vi "FuncVI-probe.vi"(5 "InstanceRef":T2, 9 "arg list":T1[](array[typedef])) -> (0 "error out":bool, 3 "result":T1)   [LabVIEW 2021]
doc: "::: CalcExpress Toolkit :::\nCopyright (c) 2000-2026 Konstantin Shifershteyn. All rights reserved."
uses:
  cetypes.llb/CalcExpress Function Argument Info.ctl
  cetypes.llb/CalcExpress Instance RefNum.ctl
panel:
  in  "max arg num":i32=4
  in  "min arg num":i32=1
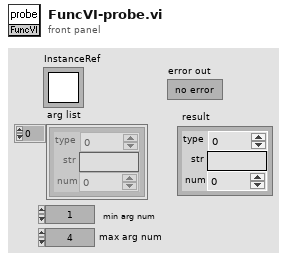
[diagram p1: front panel]
types:
  T1 = typedef "CalcExpress Function Argument Info.ctl" = cluster{"type":u32, "str":string, "num":dbl}
  T2 = typedef "CalcExpress Instance RefNum.ctl" = refnum<k1>
  T3 = cluster{"index":i32, "data type":enum32{"String", "DBL Number", "identifier", "1D Array of DBL", "2D Array of DBL", "CDB Number", "1D Array of CDB", "2D Array of CDB", "1D Array of String", "2D Array of String", "Unknown data type"}, "default num":dbl, "default str":string}[]
  T4 = cluster{"index":i32, "data type":enum32{"String", "DBL Number", "identifier", "1D Array of DBL", "2D Array of DBL", "CDB Number", "1D Array of CDB", "2D Array of CDB", "1D Array of String", "2D Array of String", "Unknown data type"}, "default num":dbl, "default str":string}
  T5 = cluster{"index":i32, "any type":i32, "default num":dbl, "default str":string}
  T6 = cluster{"data type":enum32{"String", "DBL Number", "identifier", "1D Array of DBL", "2D Array of DBL", "CDB Number", "1D Array of CDB", "2D Array of CDB", "1D Array of String", "2D Array of String", "Unknown data type"}, "str":string, "num":dbl}
  T7 = cluster{"index":i32, "data type":u32, "default num":dbl, "default str":string}[]
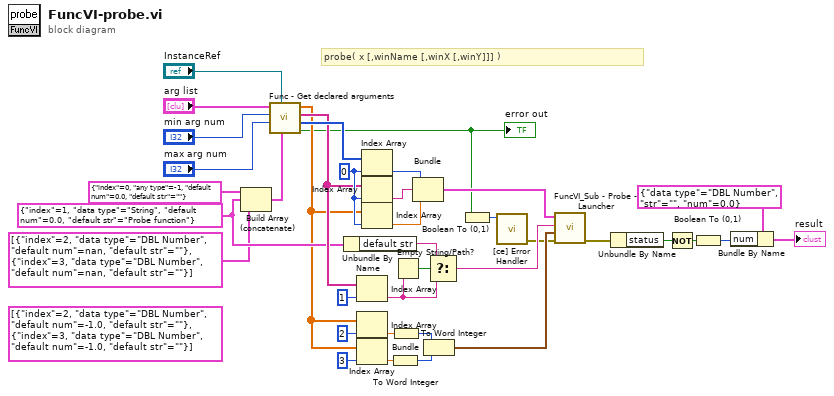
[diagram p0: block diagram]
diagram:
  (unwired) T3 [{"index"=2, "data type"=enum."DBL Number", "default num"=-1.0, "default str"=""}, {"index"=3, "data type"=enum."DBL Number", "default num"=-1.0, "default str"=""}]
  w29 = 0
  w23 = T4 {"index"=1, "data type"=enum."String", "default num"=0.0, "default str"="Probe function"} ("arg descriptor")
  # "probe( x [,winName [,winX [,winY]]] )"
  n1 = Build Array (concatenate)(T5 {"index"=0, "any type"=-1, "default num"=0.0, "default str"=""} ("arg descriptor"), w23, T3 [{"index"=2, "data type"=enum."DBL Number", "default num"=nan, "default str"=""}, {"index"=3, "data type"=enum."DBL Number", "default num"=nan, "default str"=""}]) -> (w37:T7)
  n2 = call "Func - Get declared arguments.vi"("arg descriptors"=w37, "InstanceRef"="InstanceRef", "max arg num"="max arg num", "min arg num"="min arg num", "arg list"="arg list") -> ("error out"=w1:bool, "type list"=w33:u32[], "str list"=w27:string[], "num list"=w12:dbl[])  [unwired: 3 in]
  "error out" <- w1
  n3 = Unbundle By Name(w23) -> ("default str"=w24:string)
  n4 = Index Array(array=w27, index=1) -> (element=w26:string)
  n5 = Index Array(array=w12, index=2) -> (element=w11:dbl)
  n6 = Index Array(array=w12, index=3) -> (element=w10:dbl)
  n7 = Index Array(array=w33, index=w29) -> (element=w32:u32)
  n8 = Index Array(array=w27, index=w29) -> (element=w31:string)
  n9 = Index Array(array=w12, index=w29) -> (element=w30:dbl)
  n10 = To Word Integer(number=w10) -> (16bit integer=w8:i16)
  n11 = To Word Integer(number=w11) -> (16bit integer=w9:i16)
  n12 = Empty String/Path?(string/path=w26) -> (empty?=w25:bool)
  n13 = Bundle("str"=w32, "str"=w31, "str"=w30) -> (w22:cluster{"str":u32, "str":string, "str":dbl})  [unwired: 1 in]
  n14 = Bundle(w9, w8) -> (w4:cluster{i16, i16})  [unwired: 1 in]
  n15 = Select(t=w24, s=w25, f=w26) -> (s? t:f=w21:string)
  n16 = Boolean To (0,1)(Boolean=w1) -> (0, 1=w2:i16)
  n17 = call "[ce] Error Handler.vi"("error code"=w2) -> ("error out"=w3:errorcluster)  [unwired: 9 in, 1 out]
  n18 = call "FuncVI_Sub - Probe - Launcher.vi"("error in"=w3, "left-top corner"=w4, "win name"=w21, "arg"=w22) -> ("error out"=w20:errorcluster)  [unwired: 7 in]
  n19 = Unbundle By Name(w20) -> ("status"=w19:bool)
  n20 = Not(x=w19) -> (.not. x?=w5:bool)
  n21 = Boolean To (0,1)(Boolean=w5) -> (0, 1=w18:i16)
  n22 = Bundle By Name(cluster=T6 {"data type"=enum."DBL Number", "str"="", "num"=0.0} ("opd info"), "num"=w18) -> (→"result":T6)
